vi "Make Palettes for Library.vi"() -> ()   [LabVIEW 2012, in "Palette Generation.lvlib"]
uses:
  Palette Generation.lvlib
  <vilib>/Palette API/Palette Menu/Public Type Define/Palette type.ctl
  <vilib>/Palette API/Palette Menu/Palette Menu.lvlib
panel:
  in  "All files Libraries in Directory":bool
  in  "Build Class Hierarchy":bool
  in  "Done":bool
  in  "Process":bool
  out "Progress":u8(slide) scale=0.0..100.0
  in  "Overwrite Always":bool
  in  "Library Path":path
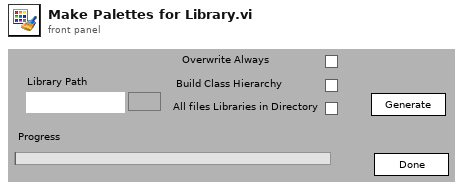
[diagram p1: front panel]
types:
  T1 = enum32{"existing file", "new file", "new or existing file", "existing dir", "new dir", "new or existing dir", "existing file (use LLBs)", "new file (use LLBs)", "new or existing file (use LLBs)", "new or existing file or directory (use LLBs)", "existing dir (use LLBs)", "new dir (use LLBs)", "new or existing dir (use LLBs)", "existing file or dir", "new file or dir", "new or existing file or dir", "existing file or dir (use LLBs)", "new file or dir (use LLBs)"}
  T2 = typedef "Palette Generation.lvlib/Palette Fiole List.ctl" = cluster{"Name":string, "Entries":cluster{string, refnum<vi>}[], "Short Name":string}
  T3 = typedef "Palette Menu.lvlib/Palette type.ctl" = i32
  T4 = typedef "Palette Menu.lvlib/Palette Data.ctl" = cluster{"display name":string, "view format":T5, "palette width":i16, "items":T6, "256 color icon":picture, "B&W color icon":picture, "help information":T8, "palette description":string, "synchronize information":T9}
  T5 = typedef "Palette Menu.lvlib/View Format.ctl" = u16
  T6 = typedef "Palette Menu.lvlib/Items.ctl" = T7[]
  T7 = typedef "Palette Menu.lvlib/Item.ctl" = cluster{"item path":path, "library path (.lvlib)":path, "use default lvlib palette":bool, "short name":string, "place VI contents":bool, "hide synchronized item":bool, "reserve spot for synch item":bool, "configure when placing VI contents":bool}
  T8 = typedef "Palette Menu.lvlib/Help Info.ctl" = cluster{"help tag":string, "help file path ":path}
  T9 = typedef "Palette Menu.lvlib/Synchronize Info.ctl" = cluster{"synchronize with directory":bool, "synchronize directory path":path}
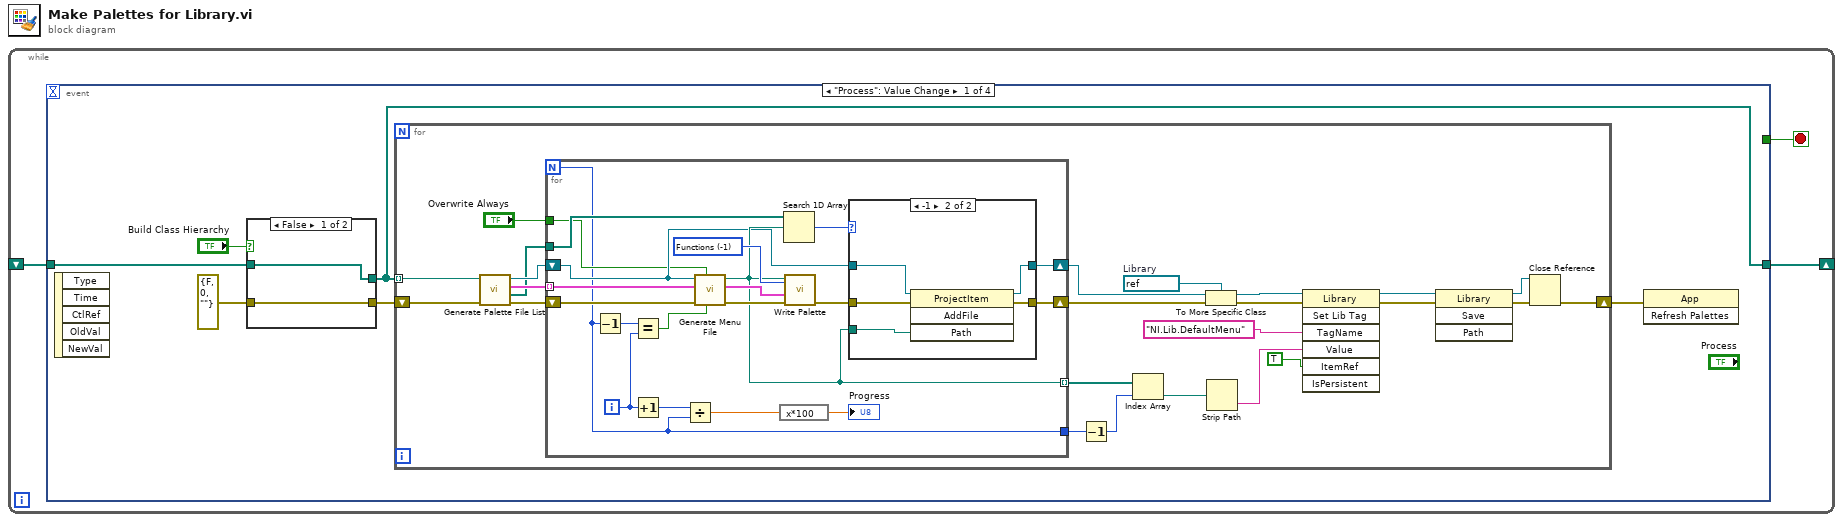
[diagram p0: block diagram]
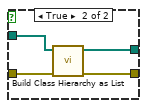
[diagram p2: hidden frame]
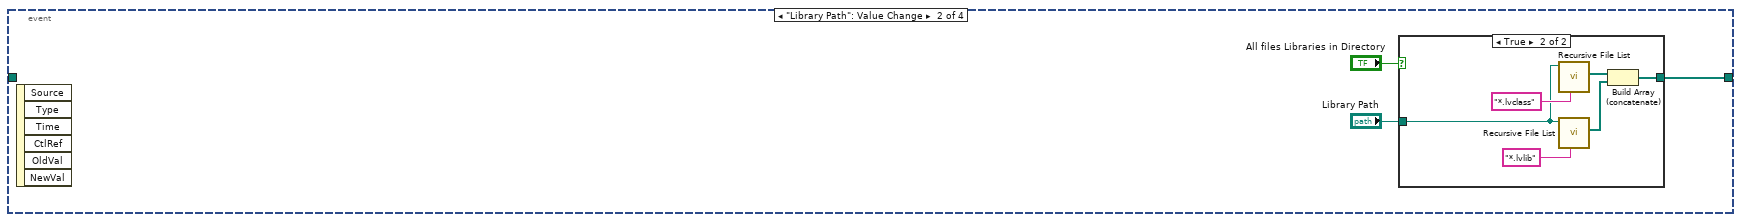
[diagram p4: hidden frame]
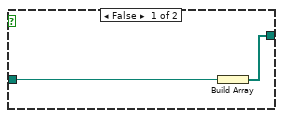
[diagram p5: hidden frame]
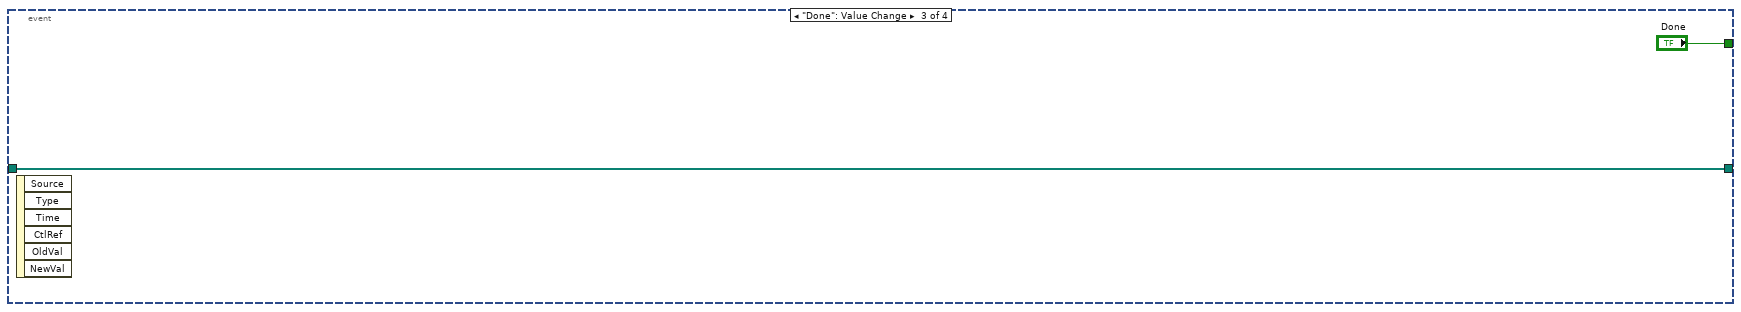
[diagram p6: hidden frame]
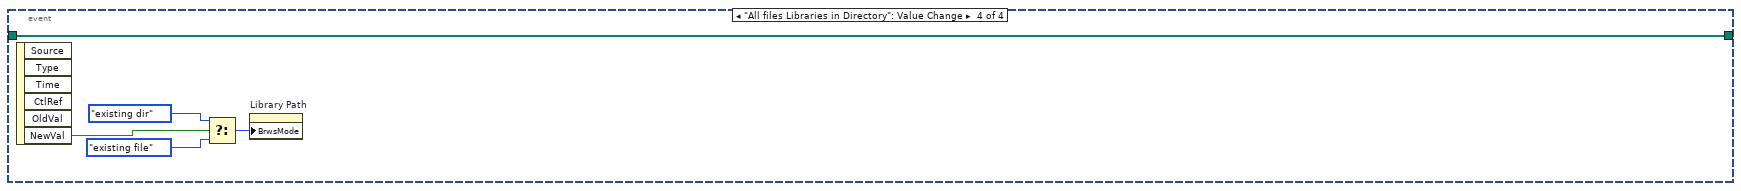
[diagram p7: hidden frame]
diagram:
  n1 = while {
    shift-right: [w2] -> _
    shift-left: _ -> [w1]
    stop <- w3 stop-if-true
    n2 = event shown="[0] \"Process\": Value Change" {
      selector: _ -> [_ _ _ _]
      dyn-events: _ -> [_ _ _ _]
      timeout: _ -> [_ _ _ _]
      tunnel: [_ _ "Done" _] -> w3
      tunnel: [w8 w68 w78 w84] -> w2
      tunnel: w1 -> [w9 _ w78 w84]
      event "Process": Value Change {
        n3 = event-data() -> ()  [unwired: 6 out]
        n4 = case shown="False" "Build Class Hierarchy" {
          tunnel: w9 -> [w11 w15]
          tunnel: [w11 w14] -> w8
          tunnel: [w10 w13] -> w5
          tunnel: errorcluster {"status"=FALSE, "code"=0, "source"=""} ("error in (no error)") -> [w10 w12]
          frame False {
          }
          frame True {
            n5 = call "Build Class Hierarchy as List.vi"("error in (no error)"=w12, "List of Class Paths"=w15) -> ("error out"=w13:errorcluster, "List of Class Paths Out"=w14:path[])  [unwired: 8 out]
          }
        }
        n6 = for {
          tunnel: w8 -> [w31] mode=indexing
          shift-right: [w29] -> w6
          shift-left: w5 -> [w30]
          w34 = refnum<vi> refnum  # Library
          n7 = call "Generate Palette File List.vi"("error in (no error)"=w30, "Library Path"=w31) -> ("error out"=w37:errorcluster, "Paths"=w33:path[], "List of Palette Files"=w39:T2[], "Library as Project item"=w38:refnum<vi>)  [unwired: 6 out]
          n8 = for {
            N -> [w40]
            tunnel: w39 -> [w59] mode=indexing
            shift-right: [w54] -> w35
            shift-left: w37 -> [w58]
            shift-right: [w53] -> w36
            shift-left: w38 -> [w49]
            tunnel: [w51] -> w25 mode=indexing
            tunnel: w33 -> [w52]
            tunnel: "Overwrite Always" -> [w47]
            tunnel: [w40] -> w23
            i -> [w43]
            w55 = T3 -1 items=["Functions"=-1, "Controls"=-2] ("palette type")
            n9 = Decrement(x=w40) -> (x-1=w44:i32)
            n10 = Equal?(x=w44, y=w43) -> (x = y?=w42:bool)
            n11 = Increment(x=w43) -> (x+1=w41:i32)
            n12 = Divide(x=w41, y=w40) -> (x/y=w46:dbl)
            n13 = call "Generate Menu File.vi"("Include Ancestor Palette ?"=w42, "Overwrite Always"=w47, "error in (no error)"=w58, "Palette Fiole List"=w59, "Library as Project item"=w49) -> ("error out"=w57:errorcluster, "palette data"=w56:T4, "Palette file path"=w51:path)  [unwired: 4 out]
            n14 = expression code="x*100"(w46) -> (→"Progress":dbl)
            n15 = Search 1D Array(1D array=w52, element=w51) -> (index of element=w50:i32)  [unwired: 1 out]
            n16 = call <vilib>:"Write Palette.vi"("error in (no error)"=w57, "palette data"=w56, "palette type"=w55, "palette path"=w51) -> ("error out"=w48:errorcluster)  [unwired: 1 in, 6 out]
            n17 = case shown="-1" w50 {
              tunnel: [w60 w66] -> w54
              tunnel: [w61 w65] -> w53
              tunnel: w51 -> [_ w64]
              tunnel: w49 -> [w61 w63]
              tunnel: w48 -> [w60 w62]
              frame 0, Default {
              }
              frame -1 {
                n18 = invoke class="ProjectItem" method="AddFile"(reference=w63, error in=w62, "Path"=w64) -> (reference out=w65:refnum<vi>, error out=w66:errorcluster)  [unwired: 1 in, 2 out]
              }
            }
          }
          n19 = Decrement(x=w23) -> (x-1=w22:i32)
          n20 = Index Array(array=w25, index=w22) -> (element=w24:path)
          n21 = To More Specific Class(target class=w34, reference=w36, error in=w35) -> (specific class reference=w21:refnum<vi>, error out=w18:errorcluster)
          n22 = Strip Path(path=w24) -> (name=w27:string)  [unwired: 1 out]
          n23 = invoke class="Library" method="Set Lib Tag"(reference=w21, error in=w18, "TagName"="NI.Lib.DefaultMenu" ("Tag Name"), "Value"=w27, "ItemRef"=TRUE ("Is Persistent")) -> (reference out=w20:refnum<vi>, error out=w17:errorcluster)  [unwired: 2 in, 5 out]
          n24 = invoke class="Library" method="Save"(reference=w20, error in=w17) -> (reference out=w19:refnum<vi>, error out=w16:errorcluster)  [unwired: 2 in, 2 out]
          n25 = Close Reference(reference=w19, error in (no error)=w16) -> (error out=w29:errorcluster)
        }
        n26 = invoke class="App" method="Refresh Palettes"(error in=w6) -> ()  [unwired: 2 in, 3 out]
      }
      event "Library Path": Value Change {
        n27 = event-data() -> ()  [unwired: 7 out]
        n28 = case shown="True" "All files Libraries in Directory" {
          tunnel: "Library Path" -> [w71 w76]
          tunnel: [w70 w72] -> w68
          frame False {
            n29 = Build Array(w71) -> (w70:path[])
          }
          frame True {
            n30 = call <vilib>:"Recursive File List.vi"("pattern"="*.lvclass", "Folder Path"=w76) -> ("All Files in Dir"=w74:path[])  [unwired: 2 in, 7 out]
            n31 = call <vilib>:"Recursive File List.vi"("pattern"="*.lvlib", "Folder Path"=w76) -> ("All Files in Dir"=w73:path[])  [unwired: 2 in, 7 out]
            n32 = Build Array (concatenate)(w74, w73) -> (w72:path[])
          }
        }
      }
      event "Done": Value Change {
        n33 = event-data() -> ()  [unwired: 7 out]
      }
      event "All files Libraries in Directory": Value Change {
        n34 = event-data() -> ("NewVal"=w80:bool)  [unwired: 6 out]
        n35 = Select(t=T1."existing dir" ("Browse Options:Selection Mode"), s=w80, f=T1."existing file" ("Browse Options:Selection Mode")) -> (s? t:f=w81:T1)
        n36 = property on="Library Path" class="Path"("BrwsMode"=w81) -> ()  [unwired: 2 in, 2 out]
      }
    }
  }
